vi "MCLB_MouseUp.vi"(8 "error in":errorcluster, 9 "Coords":T1, 10 "Button":u16, 11 "CtlRef":refnum<vi>) -> (0 "error out":errorcluster)   [LabVIEW 2021]
doc: "Changes clicked item symbol to 'select/unselect symbol'"
uses:
  <vilib>/Utility/miscctls.llb/LVPoint32TypeDef.ctl
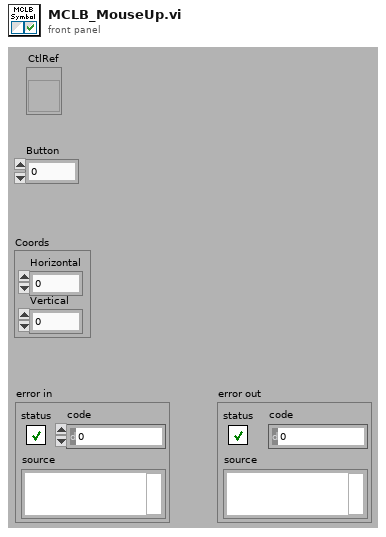
[diagram p1: front panel]
types:
  T1 = typedef "LVPoint32TypeDef.ctl" = cluster{"Horizontal":i32, "Vertical":i32}
  T2 = typedef "LVRowAndColumnTypeDef.ctl" = cluster{"Row":i32, "Column":i32}
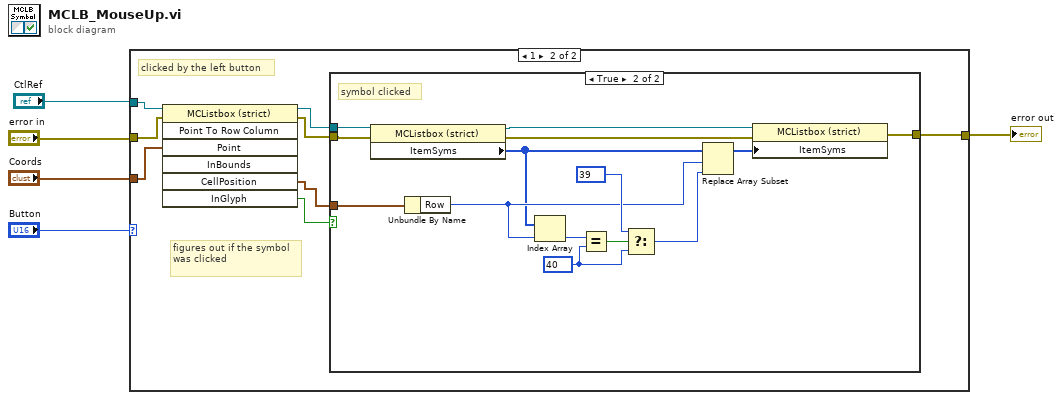
[diagram p0: block diagram]
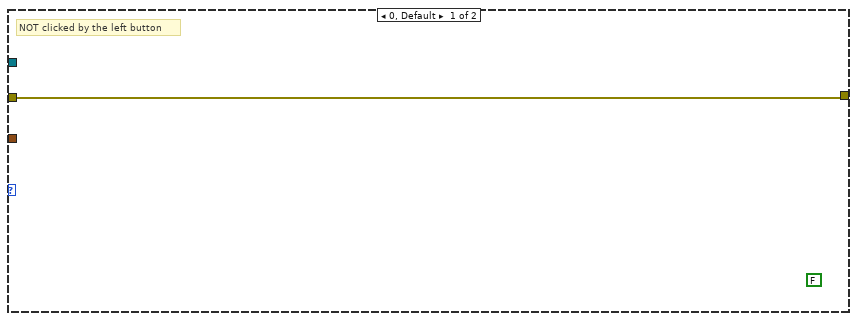
[diagram p2: hidden frame]
diagram:
  n1 = case shown="1" "Button" {
    tunnel: "Coords" -> [_ w7]
    tunnel: "error in" -> [w6 w8]
    tunnel: [w6 w14] -> w4
    tunnel: "CtlRef" -> [_ w9]
    frame 0, Default {
      (unwired) FALSE
      # "NOT clicked by the left button"
    }
    frame 1 {
      # "clicked by the left button"
      # "figures out if the symbol was clicked"
      n2 = invoke on="Invoke Node" class="MCListbox (strict)" method="Point To Row Column"(reference=w9, error in=w8, "Point"=w7) -> (reference out=w13:refnum<vi>, error out=w12:errorcluster, "CellPosition"=w11:T2, "InGlyph"=w10:bool)  [unwired: 4 in, 3 out]
      n3 = case shown="True" w10 {
        tunnel: w11 -> [_ w29]
        tunnel: w12 -> [w15 w28]
        tunnel: [w15 w25] -> w14
        tunnel: w13 -> [_ w24]
        frame False {
          # "symbol NOT clicked"
        }
        frame True {
          w19 = 40
          # "symbol clicked"
          n4 = property on="Property Node" class="MCListbox (strict)"(reference=w24, error in=w28) -> (reference out=w23:refnum<vi>, error out=w27:errorcluster, "ItemSyms"=w16:i32[])
          n5 = Unbundle By Name(w29) -> ("Row"=w17:i32)
          n6 = Index Array(array=w16, index=w17) -> (element=w22:i32)
          n7 = Equal?(x=w22, y=w19) -> (x = y?=w21:bool)
          n8 = Select(t=39, s=w21, f=w19) -> (s? t:f=w18:i32)
          n9 = Replace Array Subset(array=w16, new element=w18, index=w17) -> (w26:i32[])
          n10 = property on="Property Node" class="MCListbox (strict)"(reference=w23, error in=w27, "ItemSyms"=w26) -> (error out=w25:errorcluster)  [unwired: 1 out]
        }
      }
    }
  }
  "error out" <- w4
